vi "GetElements(Multiple).vi"(7 "Qualified Name":string, 8 "error in (no error)":errorcluster, 10 "keys":string[](array[string]), 11 "ConfigManager.Text in":refnum<class "ConfigManager.Text.lvclass">) -> (0 "error out":errorcluster, 1 "Values":string[](array[string]), 2 "Keys":string[](array[string]), 3 "ConfigManager.Text out":refnum<class "ConfigManager.Text.lvclass">, 4 "Found":bool[](array[boolean]))   [LabVIEW 2013, in "CfgManager.Text.lvlib" / "ConfigManager.Text.lvclass"]
uses:
  ConfigManager.Text.lvclass
  Query -- cluster.ctl
  Response - cluster.ctl
  ConfigManager.Text.lvclass/ConfigManager.Text.ctl
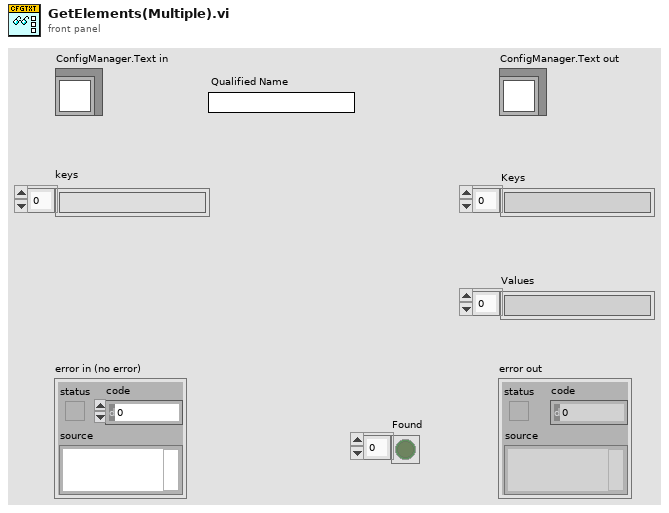
[diagram p1: front panel]
types:
  T1 = typedef "CfgManager.Text.lvlib/ConfigManager.Text.lvclass/Response - cluster.ctl" = cluster{"Section":string[], "Keys":string[], "Values":string[], "Found":bool[]}
  T2 = typedef "CfgManager.Text.lvlib/ConfigManager.Text.lvclass/Query -- cluster.ctl" = cluster{"Qualified Name":string[], "Keys":string[]}
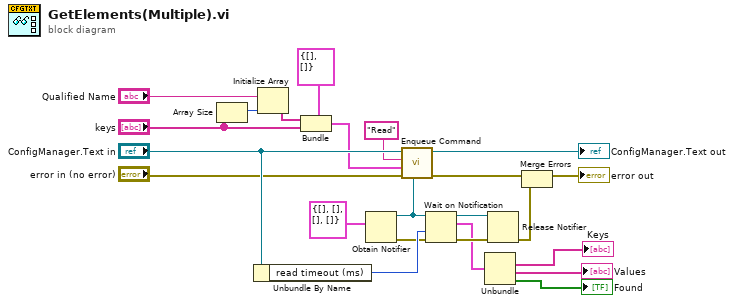
[diagram p0: block diagram]
diagram:
  n1 = Array Size(array="keys") -> (size(s)=w4:i32)
  n2 = Unbundle By Name("ConfigManager.Text in") -> ("read timeout (ms)"=w11:i32)
  n3 = Initialize Array("Qualified Name", w4) -> (w3:string[])
  n4 = Bundle(cluster=T2 {"Qualified Name"=[], "Keys"=[]} ("Query"), "Qualified Name"=w3, "Keys"="keys") -> (w5:T2)
  n5 = Obtain Notifier(notification data type=T1 {"Section"=[], "Keys"=[], "Values"=[], "Found"=[]} ("response")) -> (notifier out=w7:refnum<notifier>, error out=w10:errorcluster)  [unwired: 3 in, 1 out]
  n6 = call "Enqueue Command.vi"("query notifier"=w7, "error in (no error)"="error in (no error)", "args"=w5, "command"="Read", "ConfigManager.Text in"="ConfigManager.Text in") -> ("error out"=w2:errorcluster, "ConfigManager.Text out"=→"ConfigManager.Text out":refnum<class "ConfigManager.Text.lvclass">)  [unwired: 4 in, 1 out]
  n7 = Wait on Notification(notifier=w7, timeout in ms (-1)=w11, error in (no error)=w10) -> (notifier out=w13:refnum<notifier>, notification=w8:T1, error out=w12:errorcluster)  [unwired: 1 in, 1 out]
  n8 = Unbundle(w8) -> ("Keys"=→"Keys":string[], "Values"=→"Values":string[], "Found"=→"Found":bool[])  [unwired: 1 out]
  n9 = Release Notifier(notifier=w13, error in (no error)=w12) -> (error out=w9:errorcluster)  [unwired: 1 in, 2 out]
  n10 = Merge Errors(w2, w9) -> (→"error out":errorcluster)
